vi "Generate Key UI.vi"(11 "ID":string) -> (3 "Key":string)   [LabVIEW 2020, in "Data Viewer.lvlib"]
uses:
  Data Viewer.lvlib
panel:
  in  "Gen Key":bool
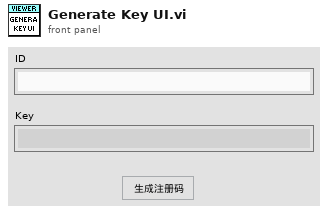
[diagram p1: front panel]
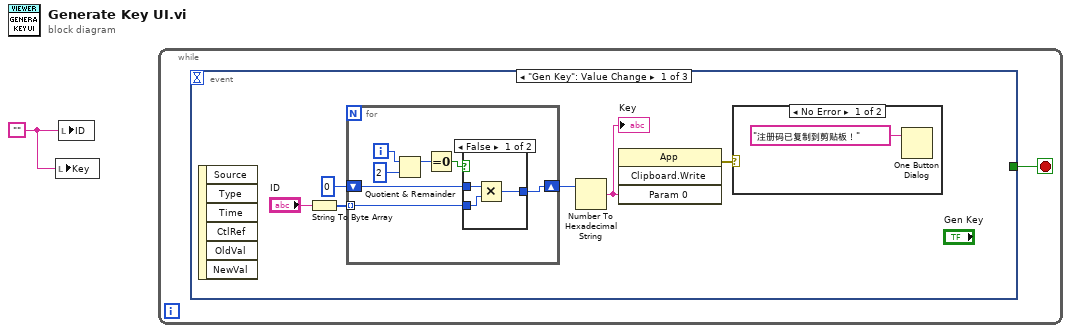
[diagram p0: block diagram]
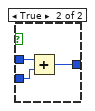
[diagram p3: hidden frame]
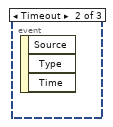
[diagram p4: hidden frame]
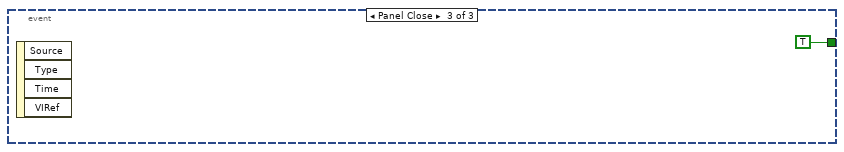
[diagram p5: hidden frame]
diagram:
  w1 = ""
  n1 = local write "Key"(w1) -> ()
  n2 = local write "ID"(w1) -> ()
  n3 = while {
    stop <- w2 stop-if-true
    n4 = event shown="[0] \"Gen Key\": Value Change" {
      selector: _ -> [_ _ _]
      dyn-events: _ -> [_ _ _]
      timeout: _ -> [_ _ _]
      tunnel: [_ _ TRUE] -> w2
      event "Gen Key": Value Change {
        n5 = event-data() -> ()  [unwired: 1 in, 6 out]
        n6 = String To Byte Array(string="ID") -> (unsigned byte array=w6:u8[])
        n7 = for {
          tunnel: w6 -> [w10] mode=indexing
          shift-right: [w15] -> w7
          shift-left: u32 0 -> [w16]
          i -> [w14]
          n8 = Quotient & Remainder(x=w14, y=2) -> (x-y*floor(x/y)=w12:i32)  [unwired: 1 out]
          n9 = Equal To 0?(x=w12) -> (x = 0?=w11:bool)
          n10 = case shown="False" w11 {
            tunnel: w16 -> [w17 w22]
            tunnel: [w19 w21] -> w15
            tunnel: w10 -> [w18 w20]
            frame False {
              n11 = Multiply(x=w17, y=w18) -> (x*y=w19:u32)
            }
            frame True {
              n12 = Add(x=w22, y=w20) -> (x+y=w21:u32)
            }
          }
        }
        n13 = Number To Hexadecimal String(2:w7) -> (0:w4:string)  [unwired: 1 in]
        "Key" <- w4
        n14 = invoke class="App" method="Clipboard.Write"("Param 0"=w4) -> (error out=w3:errorcluster)  [unwired: 3 in, 3 out]
        n15 = case shown="No Error" w3 {
          frame No Error {
            n16 = One Button Dialog(message="注册码已复制到剪贴板！") -> ()  [unwired: 1 in, 1 out]
          }
          frame Error {
          }
        }
      }
      event Timeout {
        n17 = event-data() -> ()  [unwired: 1 in, 3 out]
      }
      event Panel Close {
        n18 = event-data() -> ()  [unwired: 1 in, 4 out]
      }
    }
  }
